vi "VIH - VI Doc Editor - Shortcut Menu Handler - Picture.vi"(4 "Class Name":string, 6 "Menu Tag":string, 8 "Tree Item Tag":string, 9 "MenuRef":refnum<k9>, 10 "Terminals Tree":refnum<vi>, 11 "Event Type":T1) -> (3 "States spec":string)   [LabVIEW 2014]
doc: "::: VI Helpeks :::\nCopyright (c) 2000-2026 Konstantin Shifershteyn. All rights reserved."
uses:
  <vilib>/event_ctls.llb/lveventtype.ctl
  <vilib>/Utility/miscctls.llb/LVNodeAndColumnTypeDef.ctl
  _VIH Support Library.llb/VIH Utility - MENU - Create Menu (String).vi
panel:
  # "VI Helpeks\nCopyright (c) 2012-2026 Konstantin Shifershteyn"
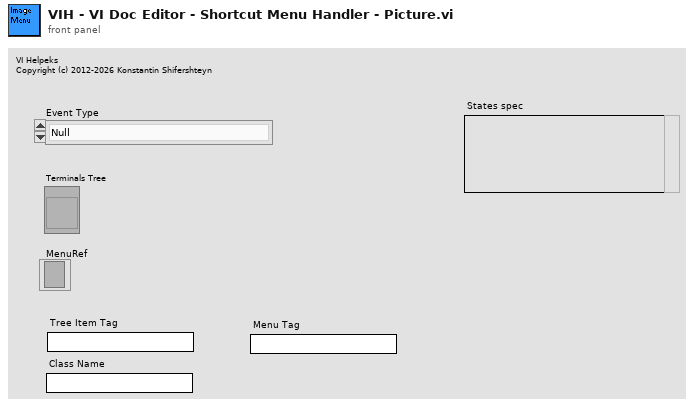
[diagram p1: front panel]
types:
  T1 = typedef "lveventtype.ctl" = enum32{"Null", "Timeout", "Annotation Menu Selection", "Annotation Menu Selection?", "App Instance Close", "App Instance Close?", "Autoscale Range Change", "Bookmark Info Change", "Cell Edit", "Cell Edit?", "Cursor Grab", "Cursor Grab?", "Cursor Menu Selection", "Cursor Menu Selection?", "Cursor Move", "Cursor Release", "Data Change", "Direction Change", "Display State Change", "Drag Ended", "Drag Enter", "Drag Leave", "Drag Over", "Drag Source Update", "Drag Starting", "Drag Starting?", "Drop", "Exec State Change", "Key Down", "Key Down?", "Key Repeat", "Key Repeat?", "Key Up", "Listbox Double Click", "Menu Activation?", "Menu Selection (App)", "Menu Selection? (App)", "Menu Selection (User)", "Mouse Down", "Mouse Down?", "Mouse Enter", "Mouse Leave", "Mouse Move", "Mouse Up", "Mouse Wheel", "NI Security User Change (App)", "Pane Size", "Panel Close", "Panel Close?", "Panel Resize", "Plot Attribute Change", "Scale Range Change", "Shortcut Menu Activation?", "Shortcut Menu Selection (App)", "Shortcut Menu Selection? (App)", "Shortcut Menu Selection (User)", "Tree Double Click", "Tree Drag", "Tree Drag?", "Tree Drop", "Tree Drop?", "Tree Item Close", "Tree Item Close?", "Tree Item Open", "Tree Item Open?", "User Event", "Value Change"}
  T2 = typedef "LVNodeAndColumnTypeDef.ctl" = cluster{"Node":string, "Column":i32}
  T3 = typedef "VIH Project Tree Typedef - Tree Refnum.ctl" = refnum<vi>
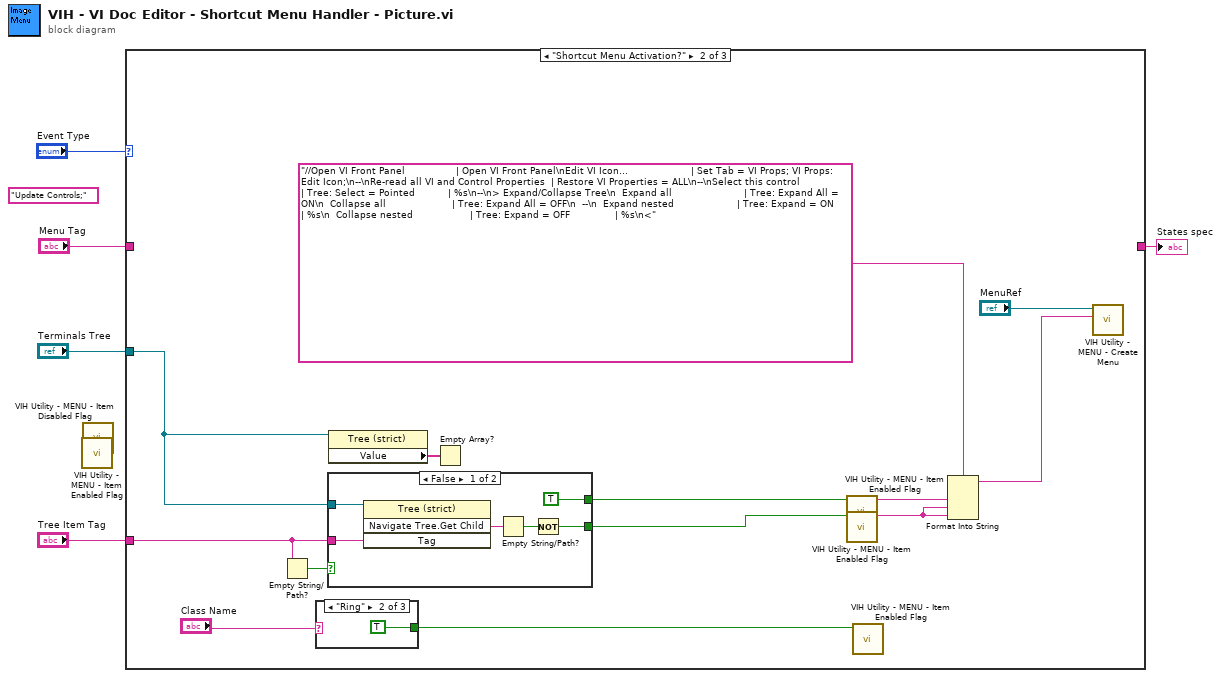
[diagram p0: block diagram]
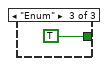
[diagram p4: hidden frame]
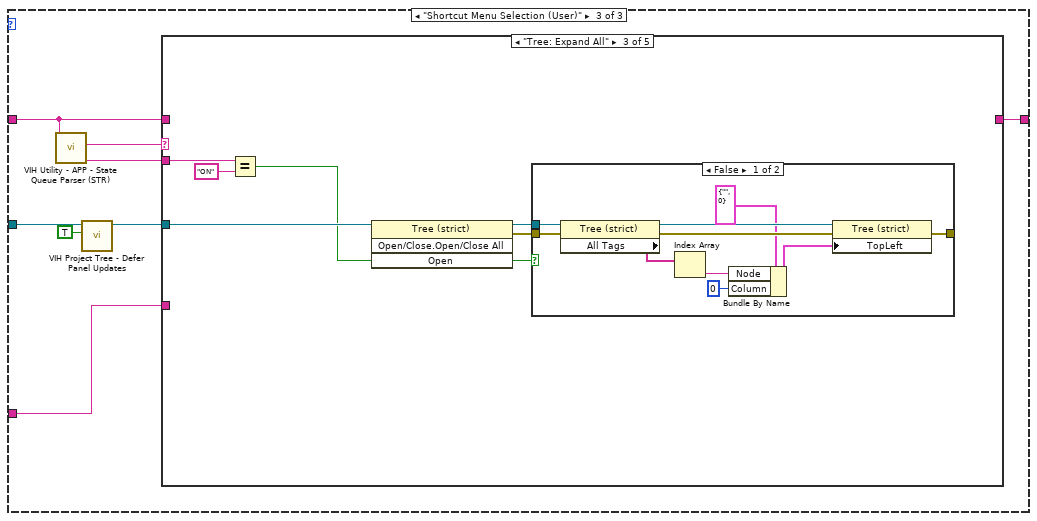
[diagram p6: hidden frame]
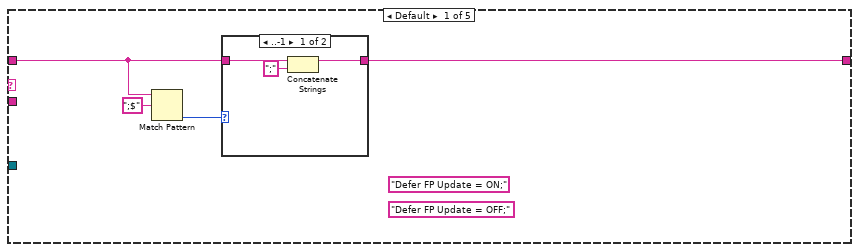
[diagram p7: hidden frame]
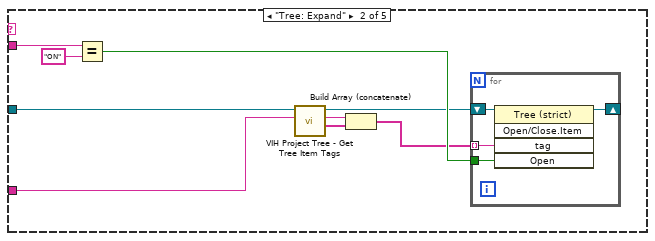
[diagram p9: hidden frame]
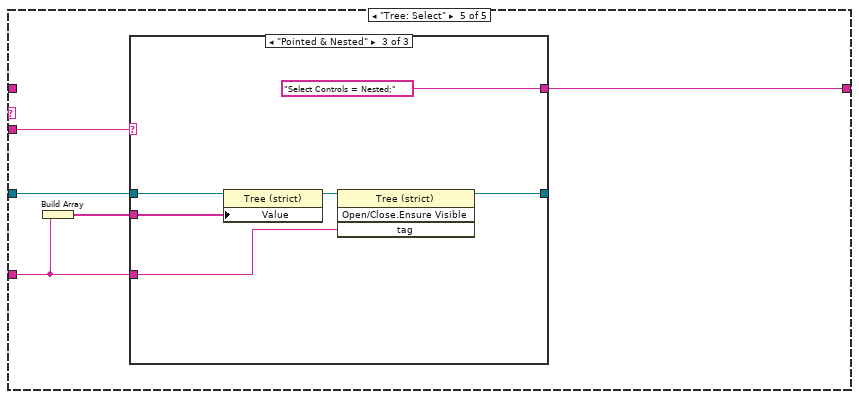
[diagram p12: hidden frame]
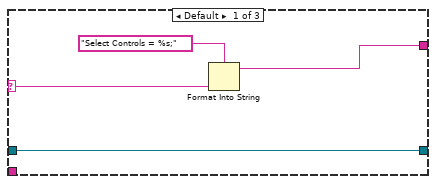
[diagram p13: hidden frame]
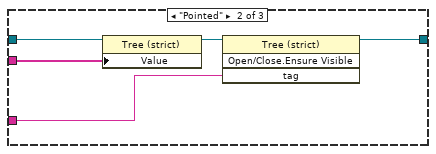
[diagram p14: hidden frame]
diagram:
  (unwired) "Update Controls;" ("Menu Tag")
  n1 = call "VIH Utility - MENU - Item Enabled Flag.vi"() -> ()  [unwired: 11 in, 1 out]
  n2 = call "VIH Utility - MENU - Item Disabled Flag.vi"() -> ()  [unwired: 11 in, 1 out]
  n3 = case shown="\"Shortcut Menu Activation?\"" "Event Type" {
    tunnel: "Terminals Tree" -> [_ w11 w28]
    tunnel: [_ _ w32] -> w3
    tunnel: "Menu Tag" -> [_ _ w33]
    tunnel: "Tree Item Tag" -> [_ w13 w30]
    frame Default {
    }
    frame "Shortcut Menu Activation?" {
      n4 = Empty String/Path?(string/path=w13) -> (empty?=w14:bool)
      n5 = case shown="\"Ring\"" "Class Name" {
        tunnel: [_ TRUE TRUE] -> w7
        frame Default {
        }
        frame "Ring" {
        }
        frame "Enum" {
        }
      }
      n6 = case shown="False" w14 {
        tunnel: [w24 _] -> w15
        tunnel: w11 -> [w23 _]
        tunnel: w13 -> [w22 _]
        tunnel: [TRUE _] -> w12
        frame False {
          n7 = invoke class="Tree (strict)" method="Navigate Tree.Get Child"(reference=w23, "Tag"=w22) -> ("Navigate Tree:Get Child"=w26:string)  [unwired: 2 in, 3 out]
          n8 = Empty String/Path?(string/path=w26) -> (empty?=w25:bool)
          n9 = Not(x=w25) -> (.not. x?=w24:bool)
        }
        frame True {
        }
      }
      n10 = property class="Tree (strict)"(reference=w11) -> ("Value"=w10:string[])  [unwired: 1 in, 2 out]
      n11 = Empty Array?(array=w10) -> ()  [unwired: 1 out]
      n12 = call "VIH Utility - MENU - Item Enabled Flag.vi"("Enable?"=w12) -> ("Disable flag"=w9:string)  [unwired: 10 in]
      n13 = call "VIH Utility - MENU - Item Enabled Flag.vi"("Enable?"=w15) -> ("Disable flag"=w6:string)  [unwired: 10 in]
      n14 = call "VIH Utility - MENU - Item Enabled Flag.vi"("Enable?"=w7) -> ()  [unwired: 10 in, 1 out]
      n15 = Format Into String(format string="//Open VI Front Panel                 | Open VI Front Panel\nEdit VI Icon...                     | Set Tab = VI Props; VI Props: Edit Icon;\n--\nRe-read all VI and Control Properties  | Restore VI Properties = ALL\n--\nSelect this control                 | Tree: Select = Pointed           | %s\n--\n> Expand/Collapse Tree\n  Expand all                        | Tree: Expand All = ON\n  Collapse all                      | Tree: Expand All = OFF\n  --\n  Expand nested                     | Tree: Expand = ON                | %s\n  Collapse nested                   | Tree: Expand = OFF               | %s\n<", w9, w6, w6) -> (resulting string=w16:string)  [unwired: 2 in, 1 out]
      n16 = call-poly "VIH Utility - MENU - Create Menu.vi"("Menu Description"=w16, "menu"="MenuRef") -> ()  [unwired: 8 in, 2 out]
    }
    frame "Shortcut Menu Selection (User)" {
      n17 = call "VIH Utility - APP - State Queue Parser (STR).vi"("input queue"=w33) -> ("state parameters"=w31:string, "state"=w34:string)  [unwired: 5 in, 2 out]
      n18 = call "VIH Project Tree - Defer Panel Updates.vi"("Defer Panel Updates (F)"=TRUE, "Project Tree"=w28) -> ("dup Project Tree"=w27:T3)  [unwired: 7 in, 2 out]
      n19 = case shown="\"Tree: Expand All\"" w34 {
        tunnel: [w35 _ _ _ w75] -> w32
        tunnel: w33 -> [w36 _ _ _ _]
        tunnel: w27 -> [_ w43 w59 _ w73]
        tunnel: w30 -> [_ w51 _ _ w74]
        tunnel: w31 -> [_ w50 w61 _ w77]
        frame Default {
          (unwired) "Defer FP Update = OFF;"
          (unwired) "Defer FP Update = ON;"
          n20 = Match Pattern(string=w36, regular expression=";$") -> (offset past match=w37:i32)  [unwired: 1 in, 3 out]
          n21 = case shown="..-1" w37 {
            tunnel: w36 -> [w41 w42]
            tunnel: [w40 w42] -> w35
            frame ..-1 {
              n22 = Concatenate Strings(w41, ";" ("string")) -> (w40:string)
            }
            frame 0.. {
            }
          }
        }
        frame "Tree: Expand" {
          n23 = Equal?(x=w50, y="ON") -> (x = y?=w48:bool)
          n24 = call "VIH Project Tree - Get Tree Item Tags.vi"("Parent Item Tag"=w51, "Project Tree"=w43) -> ("Child Item Tags"=w45:string[], "dup Parent Item Tag"=w46:string, "dup Project Tree"=w44:T3)  [unwired: 6 in, 1 out]
          n25 = Build Array (concatenate)(w46, w45) -> (w47:string[])
          n26 = for {
            tunnel: w47 -> [w54] mode=indexing
            tunnel: w48 -> [w53]
            shift-right: [w52] -> _
            shift-left: w44 -> [w55]
            n27 = invoke class="Tree (strict)" method="Open/Close.Item"(reference=w55, "tag"=w54, "Open"=w53) -> (reference out=w52:T3)  [unwired: 2 in, 4 out]
          }
        }
        frame "Tree: Expand All" {
          n28 = Equal?(x=w61, y="ON") -> (x = y?=w58:bool)
          n29 = invoke class="Tree (strict)" method="Open/Close.Open/Close All"(reference=w59, "Open"=w58) -> (reference out=w56:T3, error out=w57:errorcluster)  [unwired: 2 in, 2 out]
          n30 = case shown="False" w58 {
            tunnel: [w68 w72] -> _
            tunnel: w57 -> [w66 w72]
            tunnel: w56 -> [w65 _]
            frame False {
              n31 = property class="Tree (strict)"(reference=w65, error in=w66) -> (reference out=w64:T3, error out=w67:errorcluster, "All Tags"=w71:string[])
              n32 = Index Array(array=w71) -> (element=w70:string)  [unwired: 1 in]
              n33 = Bundle By Name(cluster=T2 {"Node"="", "Column"=0} ("Top Left Visible Cell"), "Node"=w70, "Column"=0) -> (w62:T2)
              n34 = property class="Tree (strict)"(reference=w64, error in=w67, "TopLeft"=w62) -> (error out=w68:errorcluster)  [unwired: 1 out]
            }
            frame True {
            }
          }
        }
        frame "----------------------------- 1" {
        }
        frame "Tree: Select" {
          n35 = Build Array(w74) -> (w76:string[])
          n36 = case shown="\"Pointed & Nested\"" w77 {
            selector: w77 -> [w81 _ _]
            tunnel: w73 -> [w78 w86 w92]
            tunnel: w76 -> [_ w85 w91]
            tunnel: [w79 _ "Select Controls = Nested;"] -> w75
            tunnel: w74 -> [_ w83 w88]
            tunnel: [w78 w82 w87] -> _
            frame Default {
              n37 = Format Into String(format string="Select Controls = %s;", w81) -> (resulting string=w79:string)  [unwired: 2 in, 1 out]
            }
            frame "Pointed" {
              n38 = property on="Property Node" class="Tree (strict)"(reference=w86, "Value"=w85) -> (reference out=w84:T3)  [unwired: 1 in, 1 out]
              n39 = invoke class="Tree (strict)" method="Open/Close.Ensure Visible"(reference=w84, "tag"=w83) -> (reference out=w82:T3)  [unwired: 2 in, 3 out]
            }
            frame "Pointed & Nested" {
              n40 = property on="Property Node" class="Tree (strict)"(reference=w92, "Value"=w91) -> (reference out=w89:T3)  [unwired: 1 in, 1 out]
              n41 = invoke class="Tree (strict)" method="Open/Close.Ensure Visible"(reference=w89, "tag"=w88) -> (reference out=w87:T3)  [unwired: 2 in, 3 out]
            }
          }
        }
      }
    }
  }
  "States spec" <- w3
